vi "Acquire.vi"(8 "error in (no error)":errorcluster, 11 "DAQmxDI in":refnum<class "DAQmxDI.lvclass">) -> (0 "error out":errorcluster, 3 "DAQmxDI out":refnum<class "DAQmxDI.lvclass">)   [LabVIEW 2020, in "VolatusDAQ.lvlib" / "DAQmxDI.lvclass"]
uses:
  DAQmxDI.lvclass
  DAQmxDI.lvclass/DAQmxDI.ctl
  <vilib>/DAQmx/read.llb/DAQmx Read (Digital 2D U32 NChan NSamp).vi
  <vilib>/DAQmx/miscellaneous.llb/DAQmx Fill In Error Info.vi
  VolatusData/VolatusData.lvlib
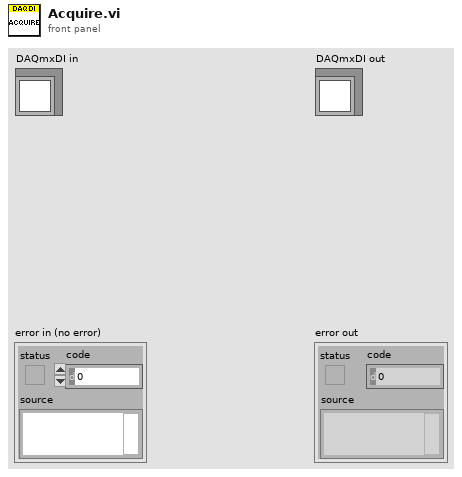
[diagram p1: front panel]
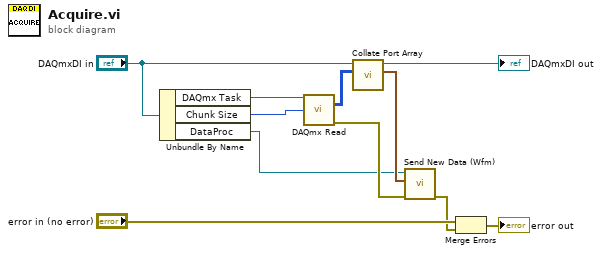
[diagram p0: block diagram]
diagram:
  n1 = Unbundle By Name("DAQmxDI in") -> ("DAQmx Task"=w9:refnum<k21>, "Chunk Size"=w1:i32, "DataProc"=w2:refnum<class "MessageQ.lvclass">)
  n2 = call-poly <vilib>:"DAQmx Read.vi"("task/channels in"=w9, "number of samples per channel"=w1) -> ("data"=w3:u32[][], "error out"=w11:errorcluster)  [unwired: 11 in, 1 out]
  n3 = call "Collate Port Array.vi"("data"=w3, "DAQmxDI in"="DAQmxDI in") -> ("Waveforms"=w4:waveform(dbl)[], "DAQmxDI out"=→"DAQmxDI out":refnum<class "DAQmxDI.lvclass">)  [unwired: 7 in, 1 out]
  n4 = call "Send New Data (Wfm).vi"("error in (no error)"=w11, "Channels"=w4, "MessageQ"=w2) -> ("error out"=w7:errorcluster)  [unwired: 8 in]
  n5 = Merge Errors("error in (no error)", w7) -> (→"error out":errorcluster)
